vi "adityam_sum_helper.vi"(1 "M factor":i32, 2 "array":dbl[](array[numeric])) -> (0 "S":dbl[](array[numeric]))   [LabVIEW 2026]
panel:
  out "P":i32
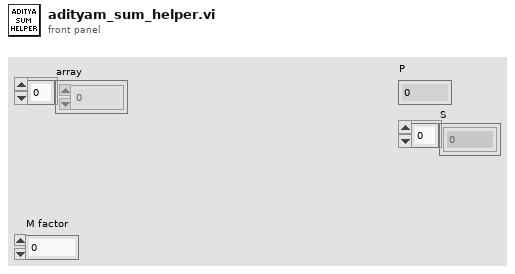
[diagram p1: front panel]
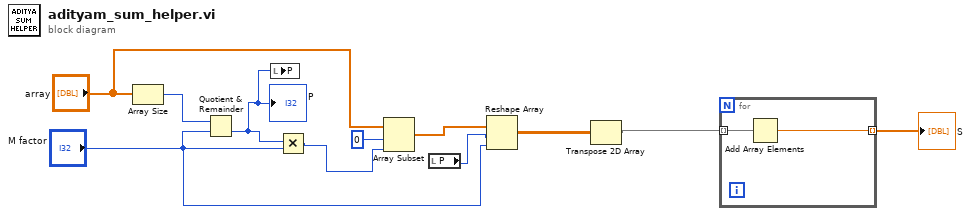
[diagram p0: block diagram]
diagram:
  n1 = Array Size(array="array") -> (size(s)=w11:i32)
  n2 = Quotient & Remainder(x=w11, y="M factor") -> (floor(x/y)=w5:i32)  [unwired: 1 out]
  "P" <- w5
  n3 = local write "P"(w5) -> ()
  n4 = Multiply(x=w5, y="M factor") -> (x*y=w9:i32)
  n5 = Array Subset(array="array", index=0, length=w9) -> (w7:dbl[])
  n6 = local read "P"() -> (w4:i32)
  n7 = Reshape Array(w7, w4, "M factor") -> (w3:dbl[][])
  n8 = Transpose 2D Array(2D array=w3) -> (transposed array=w2:dbl[][])
  n9 = for {
    tunnel: w2 -> [w13] mode=indexing
    tunnel: [w12] -> w1 mode=indexing
    n10 = Add Array Elements(numeric array=w13) -> (sum=w12:dbl)
  }
  "S" <- w1
